vi "Add Hero Image.vi"(8 "error in (no error)":errorcluster, 9 "alternateText":string, 10 "Image":path, 11 "ToastBuilder in":refnum<class "ToastBuilder.lvclass">) -> (0 "error out":errorcluster, 3 "ToastBuilder out":refnum<class "ToastBuilder.lvclass">)   [LabVIEW 2020, in "ToastNotification.lvlib" / "ToastBuilder.lvclass"]
doc: "Adds a hero image to the toast from an absolute local image path. Alternate text is optional. Skips on incoming error. The caller retains ownership of the builder."
uses:
  ToastBuilder.lvclass
  ToastBuilder.lvclass/ToastBuilder.ctl
  Toast Native/Toast Native.lvlib
  <vilib>/ErrorRing/Error Ring.xnode
  <vilib>/Utility/error.llb/Error Cluster From Error Code.vi
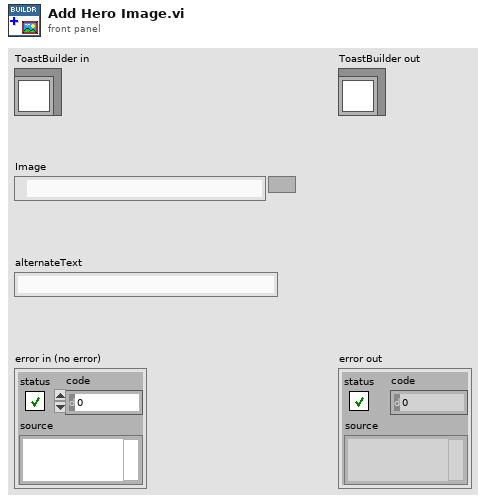
[diagram p1: front panel]
types:
  T1 = typedef "ToastNotification.lvlib/ToastBuilder.lvclass/Builder Reference.ctl" = refnum<k24>
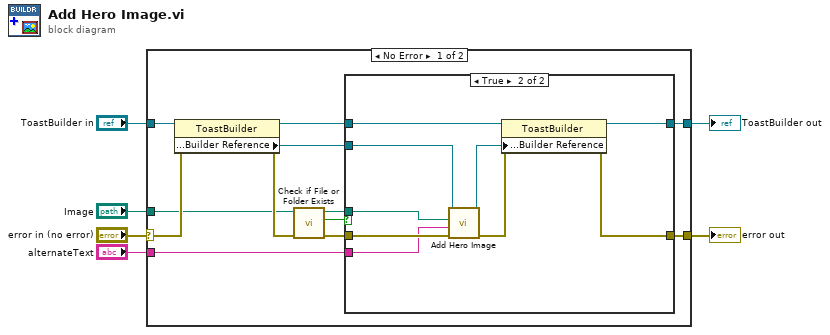
[diagram p0: block diagram]
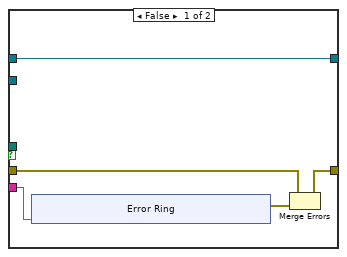
[diagram p2: hidden frame]
diagram:
  n1 = case shown="No Error" "error in (no error)" {
    selector: "error in (no error)" -> [w16 w41]
    tunnel: [w14 w41] -> w5
    tunnel: [w15 w40] -> w3
    tunnel: "ToastBuilder in" -> [w18 w40]
    tunnel: "Image" -> [w9 _]
    tunnel: "alternateText" -> [w12 _]
    frame No Error {
      n2 = property class="ToastBuilder"(reference=w18, error in=w16) -> (reference out=w17:refnum<class "ToastBuilder.lvclass">, error out=w11:errorcluster, "Public:Properties:Builder Reference"=w13:T1)
      n3 = call <vilib>:"Check if File or Folder Exists.vi"("error in (no error)"=w11, "path"=w9) -> ("error out"=w10:errorcluster, "file or folder exists?"=w7:bool, "dup path"=w8:path)  [unwired: 7 in]
      n4 = case shown="True" w7 {
        tunnel: w17 -> [w23 w39]
        tunnel: w10 -> [w21 w38]
        tunnel: [w23 w37] -> w15
        tunnel: [w19 w35] -> w14
        tunnel: w13 -> [_ w33]
        tunnel: w12 -> [w22 w32]
        tunnel: w8 -> [_ w31]
        frame False {
          n5 = xnode "Error Ring"("parameter 0"=w22) -> ("error out"=w20:errorcluster)
          n6 = Merge Errors(w21, w20) -> (w19:errorcluster)
        }
        frame True {
          n7 = call "Add Hero Image.vi"("error in (no error)"=w38, "alternateText"=w32, "Image"=w31, "reference"=w33) -> ("error out"=w36:errorcluster, "reference out"=w34:refnum<k24>)  [unwired: 6 in]
          n8 = property class="ToastBuilder"(reference=w39, error in=w36, "Public:Properties:Builder Reference"=w34) -> (reference out=w37:refnum<class "ToastBuilder.lvclass">, error out=w35:errorcluster)
        }
      }
    }
    frame Error {
    }
  }
  "error out" <- w5
  "ToastBuilder out" <- w3
